vi "Invoke Measure Logic.vi"(0 "gRPC ID in":T1, 5 "measurement plugin service in":refnum<class "Measurement Plugin Service.lvclass">, 7 "measurement service in":refnum<class "IMeasurement Service.lvclass">, 9 "measure request":T2, 11 "error in":errorcluster) -> (4 "gRPC ID out":T1, 6 "measure response":T5, 15 "error out":errorcluster)   [LabVIEW 2021, in "NI Measurement Plug-In SDK.lvlib" / "IMeasurement Service.lvclass"]
uses:
  IMeasurement Service.lvclass
  Helpers/TypeDefs/Measure Response.ctl
  gRPC/Generated APIs/ni/measurementlink/measurement/v1/RPC Messages/google_protobuf_Any.ctl
  Measurement Plugin Service/Measurement Plugin Service.lvclass
  <vilib>/gRPC/LabVIEW gRPC Library/Shared/grpcId.ctl
  Helpers/TypeDefs/Measure Request.ctl
  <vilib>/gRPC/LabVIEW gRPC Library/Shared/Any.ctl
  Helpers/TypeDefs/Pin Map Context.ctl
  Measure Call Context/Measure Call Context.lvclass
  gRPC/Generated APIs/ni/measurementlink/measurement/v1/ni.measurementlink.measurement.v1.api.lvlib
  NI Measurement Plug-In SDK.lvlib
  <vilib>/gRPC/LabVIEW gRPC Library/grpc-lvsupport-release.lvlib
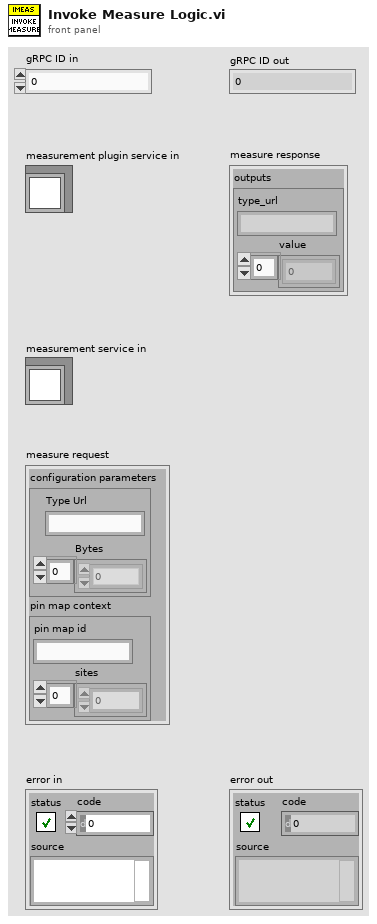
[diagram p1: front panel]
types:
  T1 = typedef "grpc-lvsupport-release.lvlib/grpcId.ctl" = u64
  T2 = typedef "NI Measurement Plug-In SDK.lvlib/Measure Request.ctl" = cluster{"configuration parameters":T3, "pin map context":T4}
  T3 = typedef "grpc-lvsupport-release.lvlib/Any.ctl" = cluster{"Type Url":string, "Bytes":u8[]}
  T4 = typedef "NI Measurement Plug-In SDK.lvlib/Pin Map Context.ctl" = cluster{"pin map id":string, "sites":i32[]}
  T5 = typedef "NI Measurement Plug-In SDK.lvlib/Measure Response.ctl" = cluster{"outputs":T6}
  T6 = typedef "ni.measurementlink.measurement.v1.api.lvlib/google_protobuf_Any.ctl" = cluster{"type_url":string, "value":u8[]}
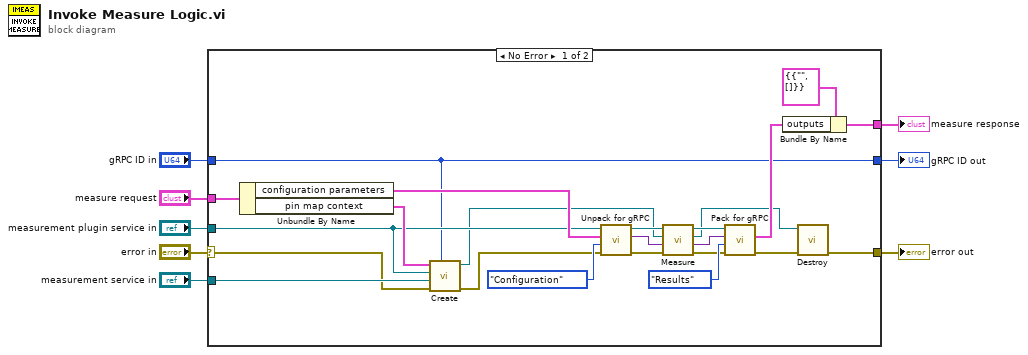
[diagram p0: block diagram]
diagram:
  n1 = case shown="No Error" "error in" {
    selector: "error in" -> [w24 w33]
    tunnel: [w9 w33] -> w7
    tunnel: [w28 _] -> w6
    tunnel: "gRPC ID in" -> [w10 w32]
    tunnel: "measurement plugin service in" -> [w21 _]
    tunnel: "measure request" -> [w27 _]
    tunnel: "measurement service in" -> [w26 _]
    tunnel: [w10 w32] -> w1
    frame No Error {
      n2 = Unbundle By Name(w27) -> ("configuration parameters"=w23:T3, "pin map context"=w31:T4)
      n3 = call "Create.vi"("gRPC server ID"=w10, "error in"=w24, "measurement service in"=w26, "measurement plugin service in"=w21, "pin map context"=w31) -> ("error out"=w20:errorcluster, "measure call context out"=w12:refnum<class "Measure Call Context.lvclass">)  [unwired: 5 in]
      n4 = call-dynamic "Unpack for gRPC.vi"("error in"=w20, "configuration / results"=enum16{"Configuration", "Results"}."Configuration" ("Configuration / Resuls (Config)"), "any"=w23, "measurement plugin service in"=w21) -> ("error out"=w19:errorcluster, "data value"=w13:variant, "measurement plugin service out"=w17:refnum<class "Measurement Plugin Service.lvclass">)  [unwired: 5 in]
      n5 = call-dynamic "Measure.vi"("error in (no error)"=w19, "measurement configuration"=w13, "measure call context in"=w12, "measurement plugin service in"=w17) -> ("error out"=w18:errorcluster, "measurement results"=w15:variant, "measure call context out"=w14:refnum<class "Measure Call Context.lvclass">, "measurement plugin service out"=w16:refnum<class "Measurement Plugin Service.lvclass">)  [unwired: 4 in]
      n6 = call-dynamic "Pack for gRPC.vi"("error in"=w18, "configuration / results"=enum16{"Configuration", "Results"}."Results" ("Configuration / Resuls (Config)"), "data value"=w15, "measurement plugin service in"=w16) -> ("error out"=w25:errorcluster, "any"=w30:T3)  [unwired: 5 in, 1 out]
      n7 = Bundle By Name(cluster=T5 {"outputs"={"type_url"="", "value"=[]}} ("measure response"), "outputs"=w30) -> (w28:T5)
      n8 = call "Destroy.vi"("error in"=w25, "measurement context in"=w14) -> ("error out"=w9:errorcluster)  [unwired: 9 in]
    }
    frame Error {
    }
  }
  "error out" <- w7
  "measure response" <- w6
  "gRPC ID out" <- w1
